vi "gainConvertPL0 (SubVI).vi"(8 "error in (no error)":errorcluster, 10 "DACin":dbl, 11 "GainIN":sgl) -> (0 "error out":errorcluster, 2 "GainOUT":sgl, 3 "DACout":dbl)   [LabVIEW 2017]
panel:
  out "FPGainOfsetPL0":sgl
  out "FPGainSlopePL0":sgl
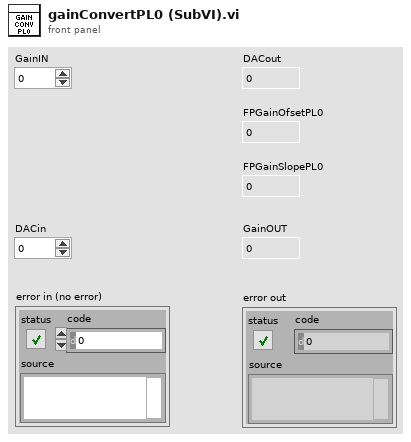
[diagram p1: front panel]
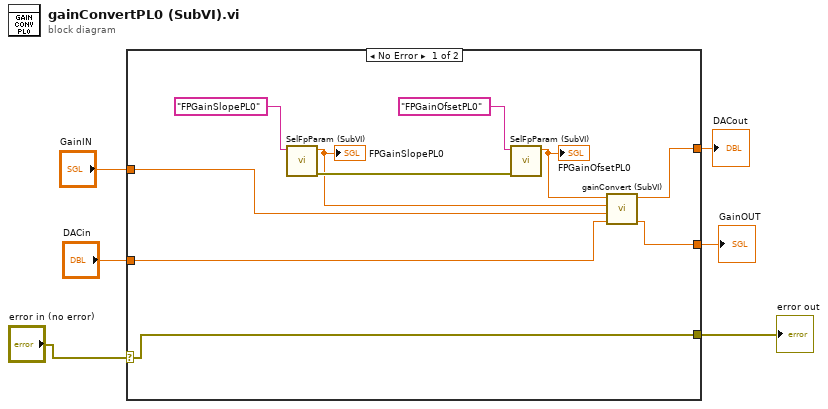
[diagram p0: block diagram]
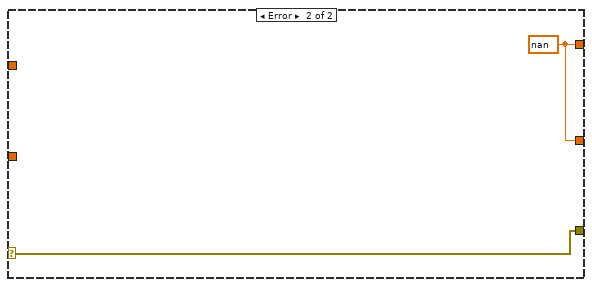
[diagram p2: hidden frame]
diagram:
  n1 = case shown="No Error" "error in (no error)" {
    selector: "error in (no error)" -> [w9 w18]
    tunnel: [w15 w17] -> w6
    tunnel: "GainIN" -> [w12 _]
    tunnel: [w9 w18] -> w3
    tunnel: [w8 w17] -> w2
    tunnel: "DACin" -> [w7 _]
    frame No Error {
      n2 = call "SelFpParam (SubVI).vi"("String"="FPGainSlopePL0") -> ("error out"=w16:errorcluster, "float number"=w14:sgl)  [unwired: 9 in]
      "FPGainSlopePL0" <- w14
      n3 = call "SelFpParam (SubVI).vi"("error in"=w16, "String"="FPGainOfsetPL0") -> ("float number"=w13:sgl)  [unwired: 8 in, 1 out]
      "FPGainOfsetPL0" <- w13
      n4 = call "gainConvert (SubVI).vi"("DACin"=w7, "GainIN"=w12, "GainSlope"=w14, "GainOffset"=w13) -> ("GainOUT"=w8:sgl, "DACout"=w15:dbl)  [unwired: 6 in]
    }
    frame Error {
      w17 = nan ("DAC")
    }
  }
  "DACout" <- w6
  "error out" <- w3
  "GainOUT" <- w2
